vi "Dispose Enumerator.vi"(8 "error in":errorcluster, 11 "Enumerator":T1) -> (0 "error out":errorcluster)   [LabVIEW 2026, in "ToastNotification.lvlib" / "Reflection DotNet.lvlib"]
doc: "Borrow an enumerator and invoke IDisposable.Dispose if its runtime type supports that interface. Attempt disposal even on an incoming error. Close acquired reflection metadata and the invocation result; merge the incoming error first. Does not close the enumerator handle: its owner must close it after this call."
uses:
  Reflection DotNet.lvlib
  Callback Object Reference.ctl
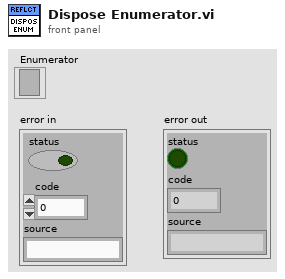
[diagram p1: front panel]
types:
  T1 = typedef "ToastNotification.lvlib/Reflection DotNet.lvlib/Callback Object Reference.ctl" = refnum<k24>
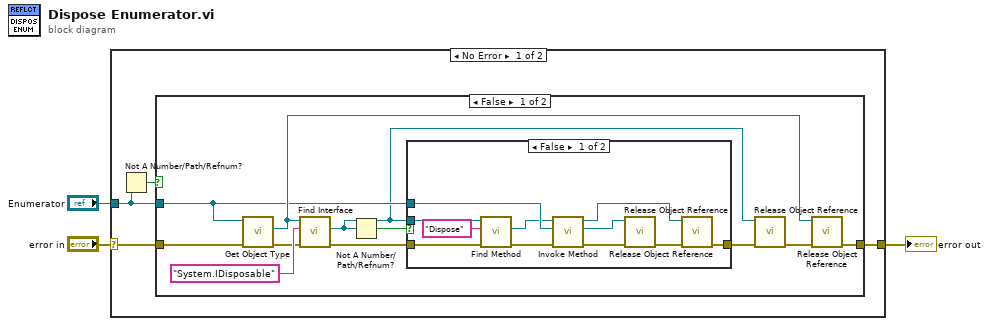
[diagram p0: block diagram]
diagram:
  n1 = case shown="No Error" "error in" {
    selector: "error in" -> [w5 w32]
    tunnel: [w7 w32] -> w3
    tunnel: "Enumerator" -> [w4 _]
    frame No Error {
      n2 = Not A Number/Path/Refnum?(number/path/refnum=w4) -> (NaN/Path/Refnum?=w6:bool)
      n3 = case shown="False" w6 {
        tunnel: w4 -> [w11 _]
        tunnel: w5 -> [w8 w31]
        tunnel: [w9 w31] -> w7
        frame False {
          n4 = call "Get Object Type.vi"("error in (no error)"=w8, "Object in"=w11) -> ("error out"=w13:errorcluster, "Object Type"=w12:refnum<k24>)  [unwired: 7 in, 1 out]
          n5 = call "Find Interface.vi"("error in (no error)"=w13, "Interface Name"="System.IDisposable", "Object Type in"=w12) -> ("error out"=w15:errorcluster, "Interface Type"=w10:refnum<k24>)  [unwired: 6 in, 1 out]
          n6 = Not A Number/Path/Refnum?(number/path/refnum=w10) -> (NaN/Path/Refnum?=w16:bool)
          n7 = case shown="False" w16 {
            tunnel: w11 -> [w22 _]
            tunnel: w10 -> [w21 _]
            tunnel: w15 -> [w23 w30]
            tunnel: [w29 w30] -> w17
            frame False {
              n8 = call "Find Method.vi"("error in (no error)"=w23, "Method Name"="Dispose", "Declaring Type in"=w21) -> ("error out"=w25:errorcluster, "Method Info"=w20:refnum<k24>)  [unwired: 6 in, 1 out]
              n9 = call "Invoke Method.vi"("error in (no error)"=w25, "Target Object"=w22, "Method Info in"=w20) -> ("error out"=w27:errorcluster, "Return Value"=w26:refnum<k24>, "Method Info out"=w19:refnum<k24>)  [unwired: 6 in]
              n10 = call "Release Object Reference.vi"("error in"=w27, "object"=w26) -> ("error out"=w28:errorcluster)  [unwired: 9 in]
              n11 = call "Release Object Reference.vi"("error in"=w28, "object"=w19) -> ("error out"=w29:errorcluster)  [unwired: 9 in]
            }
            frame True {
            }
          }
          n12 = call "Release Object Reference.vi"("error in"=w17, "object"=w10) -> ("error out"=w18:errorcluster)  [unwired: 9 in]
          n13 = call "Release Object Reference.vi"("error in"=w18, "object"=w12) -> ("error out"=w9:errorcluster)  [unwired: 9 in]
        }
        frame True {
        }
      }
    }
    frame Error {
    }
  }
  "error out" <- w3
